vi "Func - Cut _Indirect_Func_.vi"(4 "FuncVI List":string) -> (1 "FuncVI List out":string)   [LabVIEW 2021]
doc: "::: CalcExpress Toolkit :::\nCopyright (c) 2000-2026 Konstantin Shifershteyn. All rights reserved."
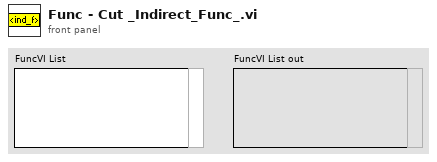
[diagram p1: front panel]
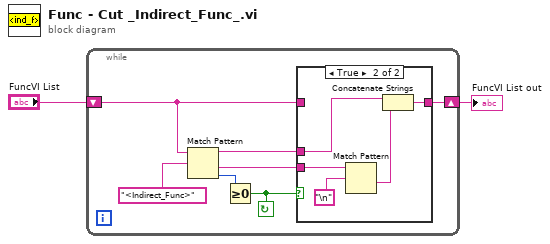
[diagram p0: block diagram]
diagram:
  n1 = while {
    shift-left: "FuncVI List" -> [w6]
    shift-right: [w5] -> w1
    stop <- w7 continue-if-true
    n2 = Match Pattern(string=w6, regular expression="<Indirect_Func>") -> (before substring=w3:string, after substring=w4:string, offset past match=w8:i32)  [unwired: 1 in, 1 out]
    n3 = Greater Or Equal To 0?(x=w8) -> (x >= 0?=w7:bool)
    n4 = case shown="True" w7 {
      tunnel: [w10 w11] -> w5
      tunnel: w6 -> [w10 _]
      tunnel: w4 -> [_ w15]
      tunnel: w3 -> [_ w12]
      frame False {
      }
      frame True {
        n5 = Match Pattern(string=w15, regular expression="\n") -> (after substring=w13:string)  [unwired: 1 in, 3 out]
        n6 = Concatenate Strings(w12, w13) -> (w11:string)
      }
    }
  }
  "FuncVI List out" <- w1
